vi "cmbBox Change List and Set Value.vi"(8 "error in (no error)":errorcluster, 9 "Current(\"\")":string, 10 "Strings []":string[](array[string]), 11 "cmbBox":refnum<vi>) -> (0 "error out":errorcluster, 3 "cmbBox(dup)":refnum<vi>)   [LabVIEW 2017, in "csm-ui-support.lvlib"]
uses:
  csm-ui-support.lvlib
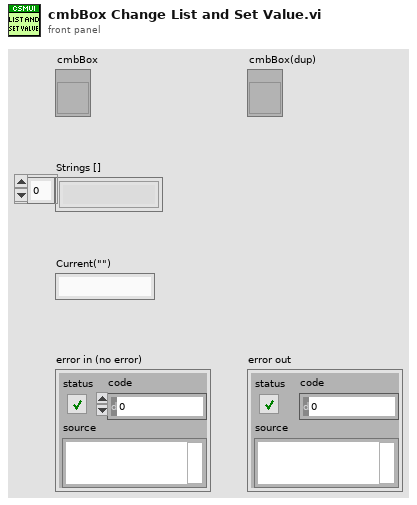
[diagram p1: front panel]
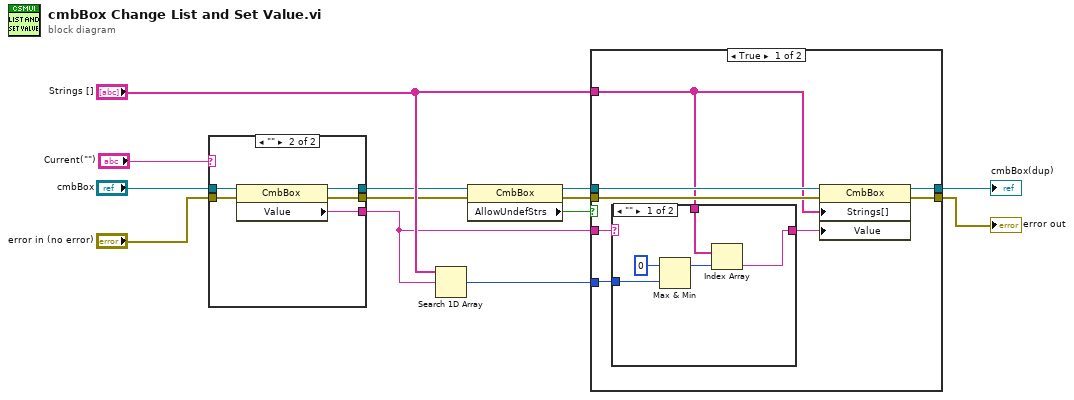
[diagram p0: block diagram]
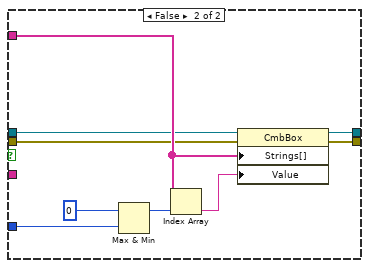
[diagram p3: hidden frame]
diagram:
  n1 = case shown="\"\"" "Current(\"\")" {
    selector: "Current(\"\")" -> [w14 _]
    tunnel: [w14 w21] -> w1
    tunnel: [w16 w20] -> w6
    tunnel: [w15 w19] -> w5
    tunnel: "cmbBox" -> [w15 w18]
    tunnel: "error in (no error)" -> [w16 w17]
    frame Default {
    }
    frame "" {
      n2 = property on="Property Node" class="CmbBox"(reference=w18, error in=w17) -> (reference out=w19:refnum<vi>, error out=w20:errorcluster, "Value"=w21:string)
    }
  }
  n3 = Search 1D Array(1D array="Strings []", element=w1) -> (index of element=w11:i32)  [unwired: 1 in]
  n4 = property on="Property Node" class="CmbBox"(reference=w5, error in=w6) -> (reference out=w3:refnum<vi>, error out=w4:errorcluster, "AllowUndefStrs"=w2:bool)
  n5 = case shown="True" w2 {
    tunnel: "Strings []" -> [w22 w44]
    tunnel: w11 -> [w23 w43]
    tunnel: [w29 w39] -> w9
    tunnel: [w28 w38] -> w8
    tunnel: w4 -> [w27 w37]
    tunnel: w3 -> [w26 w36]
    tunnel: w1 -> [w25 _]
    frame True {
      n6 = case shown="\"\"" w25 {
        selector: w25 -> [_ w35]
        tunnel: [w30 w35] -> w24
        tunnel: w23 -> [w32 _]
        tunnel: w22 -> [w31 _]
        frame "" {
          n7 = Max & Min(x=0, y=w32) -> (max(x,y)=w34:i32)  [unwired: 1 out]
          n8 = Index Array(array=w31, index=w34) -> (element=w30:string)
        }
        frame Default {
        }
      }
      n9 = property on="Property Node" class="CmbBox"(reference=w26, error in=w27, "Strings[]"=w22, "Value"=w24) -> (reference out=w29:refnum<vi>, error out=w28:errorcluster)
    }
    frame False {
      n10 = Max & Min(x=0, y=w43) -> (max(x,y)=w40:i32)  [unwired: 1 out]
      n11 = Index Array(array=w44, index=w40) -> (element=w42:string)
      n12 = property on="Property Node" class="CmbBox"(reference=w36, error in=w37, "Strings[]"=w44, "Value"=w42) -> (reference out=w39:refnum<vi>, error out=w38:errorcluster)
    }
  }
  "cmbBox(dup)" <- w9
  "error out" <- w8
